vi "FuncVI_Sub - Enter Number Dialog.vi"(6 "integer?":bool, 8 "maximum":dbl=inf, 9 "minimum":dbl=-inf, 10 "Default Value":dbl, 11 "message":string) -> (2 "value out":dbl format="%.2f")   [LabVIEW 2021]
doc: "::: CalcExpress Toolkit :::\nCopyright (c) 2000-2026 Konstantin Shifershteyn. All rights reserved."
panel:
  in  "value int":i32 caption="value" min=-1 max=1
  in  "precision":u8
  in  "format":u8(ring) items=["Decimal", "Scientific", "Engineering", "Binary", "Octal", "Hexadecimal", "Relative Time", "Date and Time", "SI"]
  in  "cancel":bool
  in  "ok":bool
  in  "value dbl":dbl caption="value" min=-1.0 max=1.0
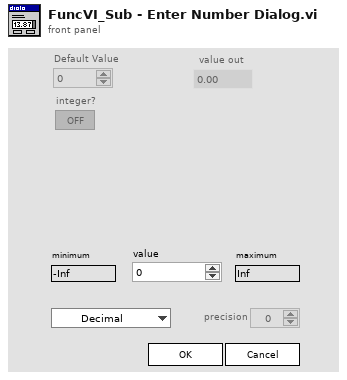
[diagram p1: front panel]
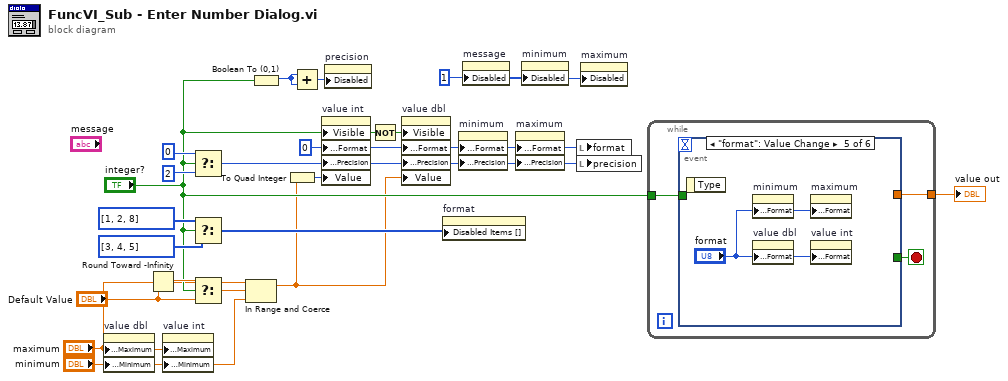
[diagram p0: block diagram]
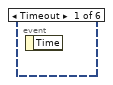
[diagram p2: hidden frame]
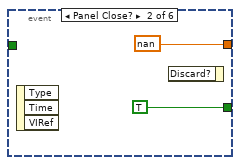
[diagram p3: hidden frame]
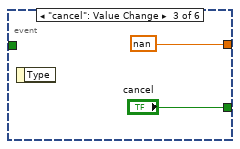
[diagram p4: hidden frame]
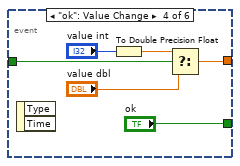
[diagram p5: hidden frame]
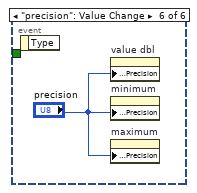
[diagram p6: hidden frame]
diagram:
  w9 = u8 0 ("Format & Precision:Format")
  w20 = u8 1 ("Disabled")
  n1 = property on="value dbl" class="DigNum (strict)"("Data Entry Limits:Maximum"="maximum", "Data Entry Limits:Minimum"="minimum") -> ()  [unwired: 2 in, 2 out]
  n2 = Round Toward -Infinity(1:"Default Value") -> (0:w13:dbl)
  n3 = property on="value int" class="DigNum (strict)"("Data Entry Limits:Maximum"="maximum", "Data Entry Limits:Minimum"="minimum") -> ()  [unwired: 2 in, 2 out]
  n4 = Select(t=u8 0 ("Format & Precision:Precision"), s="integer?", f=u8 2 ("Format & Precision:Precision")) -> (s? t:f=w19:u8)
  n5 = Select(t=i32[] [1, 2, 8] ("Disabled Items []"), s="integer?", f=i32[] [3, 4, 5] ("Disabled Items []")) -> (s? t:f=w14:i32[])
  n6 = Select(t=w13, s="integer?", f="Default Value") -> (s? t:f=w6:dbl)
  n7 = In Range and Coerce(upper limit="maximum", x=w6, lower limit="minimum") -> (coerced(x)=w1:dbl)  [unwired: 1 out]
  n8 = Boolean To (0,1)(Boolean="integer?") -> (0, 1=w10:i16)
  n9 = To Quad Integer(1:w1) -> (0:w2:i64)
  n10 = Add(x=w10, y=w10) -> (x+y=w11:i16)
  n11 = property on="value int" class="DigNum (strict)"("Visible"="integer?", "Display Format:Format"=w9, "Display Format:Precision"=w19, "Value"=w2) -> ()  [unwired: 2 in, 2 out]
  n12 = property on="precision" class="DigNum (strict)"("Disabled"=w11) -> ()  [unwired: 2 in, 2 out]
  n13 = Not(x="integer?") -> (.not. x?=w8:bool)
  n14 = property on="value dbl" class="DigNum (strict)"("Visible"=w8, "Display Format:Format"=w9, "Display Format:Precision"=w19, "Value"=w1) -> ()  [unwired: 2 in, 2 out]
  n15 = property on="format" class="Ring (strict)"("Disabled Items []"=w14) -> ()  [unwired: 2 in, 2 out]
  n16 = property on="minimum" class="DigNum (strict)"("Display Format:Format"=w9, "Display Format:Precision"=w19) -> ()  [unwired: 2 in, 2 out]
  n17 = property on="message" class="Str"("Disabled"=w20) -> ()  [unwired: 2 in, 2 out]
  n18 = property on="maximum" class="DigNum (strict)"("Display Format:Format"=w9, "Display Format:Precision"=w19) -> ()  [unwired: 2 in, 2 out]
  n19 = property on="minimum" class="DigNum (strict)"("Disabled"=w20) -> ()  [unwired: 2 in, 2 out]
  n20 = local write "format"(w9) -> ()
  n21 = local write "precision"(w19) -> ()
  n22 = property on="maximum" class="DigNum (strict)"("Disabled"=w20) -> ()  [unwired: 2 in, 2 out]
  n23 = while {
    tunnel: [w22] -> w12
    tunnel: "integer?" -> [w21]
    stop <- w23 stop-if-true
    n24 = event shown="[4] \"format\": Value Change" {
      selector: _ -> [_ _ _ _ _ _]
      dyn-events: _ -> [_ _ _ _ _ _]
      timeout: _ -> [_ _ _ _ _ _]
      tunnel: [_ TRUE "cancel" "ok" _ _] -> w23
      tunnel: [_ nan ("f") nan ("f") w29 _ _] -> w22
      tunnel: w21 -> [_ _ _ w32 _ _]
      event Timeout {
        n25 = event-data() -> ()  [unwired: 1 in, 1 out]
      }
      event Panel Close? {
        n26 = event-data() -> ()  [unwired: 1 in, 3 out]
        n27 = event-data ("Event Filter Node")() -> ()  [unwired: 2 in, 1 out]
      }
      event "cancel": Value Change {
        n28 = event-data() -> ()  [unwired: 1 in, 1 out]
      }
      event "ok": Value Change {
        n29 = event-data() -> ()  [unwired: 1 in, 2 out]
        n30 = To Double Precision Float(number="value int") -> (double precision float=w28:dbl)
        n31 = Select(t=w28, s=w32, f="value dbl") -> (s? t:f=w29:dbl)
      }
      event "format": Value Change {
        n32 = event-data() -> ()  [unwired: 1 in, 1 out]
        n33 = property on="minimum" class="DigNum (strict)"("Display Format:Format"="format") -> ()  [unwired: 2 in, 2 out]
        n34 = property on="value dbl" class="DigNum (strict)"("Display Format:Format"="format") -> ()  [unwired: 2 in, 2 out]
        n35 = property on="maximum" class="DigNum (strict)"("Display Format:Format"="format") -> ()  [unwired: 2 in, 2 out]
        n36 = property on="value int" class="DigNum (strict)"("Display Format:Format"="format") -> ()  [unwired: 2 in, 2 out]
      }
      event "precision": Value Change {
        n37 = event-data() -> ()  [unwired: 1 in, 1 out]
        n38 = property on="value dbl" class="DigNum (strict)"("Display Format:Precision"="precision") -> ()  [unwired: 2 in, 2 out]
        n39 = property on="minimum" class="DigNum (strict)"("Display Format:Precision"="precision") -> ()  [unwired: 2 in, 2 out]
        n40 = property on="maximum" class="DigNum (strict)"("Display Format:Precision"="precision") -> ()  [unwired: 2 in, 2 out]
      }
    }
  }
  "value out" <- w12
